vi "Module Cleanup.vi"(8 "error in (no error)":errorcluster, 11 "Volatus Core in":refnum<class "Volatus Core.lvclass">) -> (0 "error out":errorcluster, 3 "Volatus Core out":refnum<class "Volatus Core.lvclass">)   [LabVIEW 2020, in "Volatus.lvlib" / "Volatus Core.lvclass"]
uses:
  Volatus Core.lvclass
  Volatus Core.lvclass/Volatus Core.ctl
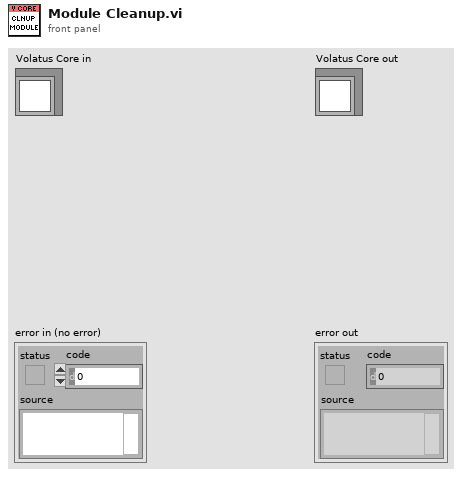
[diagram p1: front panel]
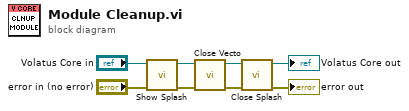
[diagram p0: block diagram]
diagram:
  n1 = call "Show Splash.vi"("error in (no error)"="error in (no error)", "Volatus Core in"="Volatus Core in") -> ("error out"=w6:errorcluster, "Volatus Core out"=w4:refnum<class "Volatus Core.lvclass">)  [unwired: 8 in]
  n2 = call "Close Vecto.vi"("error in (no error)"=w6, "Volatus Core in"=w4) -> ("error out"=w7:errorcluster, "Volatus Core out"=w2:refnum<class "Volatus Core.lvclass">)  [unwired: 8 in]
  n3 = call "Close Splash.vi"("error in (no error)"=w7, "Volatus Core in"=w2) -> ("error out"=→"error out":errorcluster, "Volatus Core out"=→"Volatus Core out":refnum<class "Volatus Core.lvclass">)  [unwired: 8 in]
